vi "Create Runtime.vi"(8 "error in (no error)":errorcluster, 11 "CIF_Iceoryx_PCAP_Universal in":refnum<class "CIF_Iceoryx_PCAP_Universal.lvclass">) -> (0 "error out":errorcluster, 3 "CIF_Iceoryx_PCAP_Universal out":refnum<class "CIF_Iceoryx_PCAP_Universal.lvclass">)   [LabVIEW 2021, in "CIF_Iceoryx_PCAP_Universal.lvclass"]
doc: "To support reconfiguration for different sizes or queue depths, the publisher will register but not create the underlying Iceoryx FIFO. Instead the creation is delayed and is created at run-time. This function is called for each channel on prepare and when a subscriber connects."
uses:
  CIF_Iceoryx_PCAP_Universal.lvclass
  D:/dev/Packages/CIF_Channels_Core/src/CIFChannels/CIFChannels.lvclass
  CIFChannels/CIFChannels.lvclass/CIFChannels.ctl
  ChannelCommon/typedef/Direction.ctl
  ChannelCommon/typedef/Channel State.ctl
  CIF_Iceoryx_PCAP_Universal.lvclass/CIF_Iceoryx_PCAP_Universal.ctl
  <vilib>/CIF Foundation/CIF Iceoryx/typedef/CIF Pcap Publisher Configuration.ctl
  CIFChannels/Accessors/Write Channel State.vi
  CIFChannels/Accessors/Read Name.vi
  CIFChannels/Accessors/Read Direction.vi
  CIFChannels/Accessors/Read Channel State.vi
  <vilib>/CIF Foundation/CIF Iceoryx/SubVIs/Get Path.vi
  <vilib>/CIF Foundation/CIF Iceoryx/SubVIs/Convert Error.vi
  <vilib>/CIF Foundation/CIF Iceoryx/SubVIs/Add Error.vi
  <vilib>/CIF Foundation/CIF Iceoryx/Refnum/CIF Publisher to Refnum.vi
  <vilib>/Utility/error.llb/Trim Whitespace.vi
  <vilib>/CIF Foundation/CIF Iceoryx/SubVIs/Add Error Core.vi
  <vilib>/CIF Foundation/CIF Iceoryx/SubVIs/Convert Error Core.vi
  <vilib>/CIF Foundation/CIF Iceoryx/Iceoryx.lvlib
  ChannelCommon/ChannelCommon.lvlib
  Iceorxy Utilities/Iceoryx Channel Utilities.lvlib
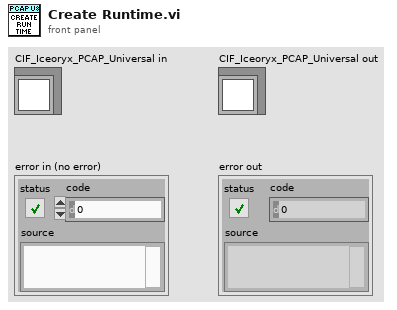
[diagram p1: front panel]
types:
  T1 = typedef "ChannelCommon.lvlib/Direction.ctl" = enum8{"Publisher", "Subscriber"}
  T2 = typedef "ChannelCommon.lvlib/Channel State.ctl" = enum8{"Creating", "Disconnected", "Connecting", "Connected", "Destroyed"}
  T3 = typedef "Iceoryx.lvlib/CIF Pcap Publisher Configuration.ctl" = cluster{"Name":string, "Topic":string, "Link Type":u32, "Descriptor":string, "Max Bytes":u32, "Best Effort Subscribers":u32, "Backpressure Subscribers":u32, "Best Effort Queue Depth":u32, "Backpressure Queue Depth":u32}
  T4 = typedef "Iceoryx.lvlib/CIF Publisher Refnum.ctl" = cluster{"refnum":u64, "CIF Pub":enum8{"cifpub"}}
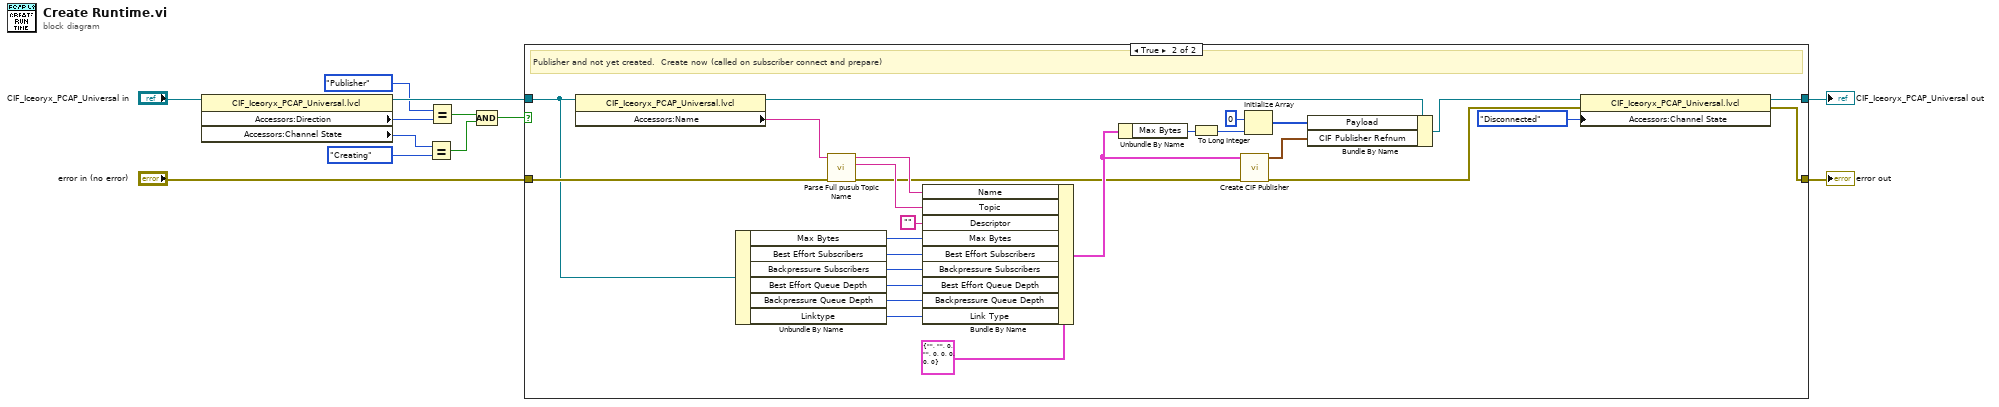
[diagram p0: block diagram]
diagram:
  n1 = property class="CIF_Iceoryx_PCAP_Universal.lvcl"(reference="CIF_Iceoryx_PCAP_Universal in") -> (reference out=w8:refnum<class "CIF_Iceoryx_PCAP_Universal.lvclass">, "Accessors:Direction"=w5:T1, "Accessors:Channel State"=w7:T2)  [unwired: 1 in, 1 out]
  n2 = Equal?(x=w7, y=Channel_State."Creating") -> (x = y?=w3:bool)
  n3 = Equal?(x=Direction."Publisher", y=w5) -> (x = y?=w2:bool)
  n4 = Compound Arithmetic op=AND(w2, w3) -> (w1:bool)
  n5 = case shown="True" w1 {
    tunnel: [w14 w32] -> w12
    tunnel: [w13 w31] -> w11
    tunnel: "error in (no error)" -> [w13 w23]
    tunnel: w8 -> [w14 w15]
    frame False {
    }
    frame True {
      # "Publisher and not yet created.  Create now (called on subscriber connect and prepare)"
      n6 = property class="CIF_Iceoryx_PCAP_Universal.lvcl"(reference=w15) -> (reference out=w25:refnum<class "CIF_Iceoryx_PCAP_Universal.lvclass">, "Accessors:Name"=w24:string)  [unwired: 1 in, 1 out]
      n7 = Unbundle By Name(w15) -> ("Max Bytes"=w22:u32, "Best Effort Subscribers"=w27:u32, "Backpressure Subscribers"=w26:u32, "Best Effort Queue Depth"=w21:u32, "Backpressure Queue Depth"=w20:u32, "Linktype"=w19:u32)
      n8 = call "Parse Full pusub Topic Name.vi"("error in"=w23, "Full pubsub Topic Name"=w24) -> ("error out"=w16:errorcluster, "Topic"=w28:string, "Plugin name"=w29:string)  [unwired: 7 in]
      n9 = Bundle By Name(cluster=T3 {"Name"="", "Topic"="", "Link Type"=0, "Descriptor"="", "Max Bytes"=0, "Best Effort Subscribers"=0, "Backpressure Subscribers"=0, "Best Effort Queue Depth"=0, "Backpressure Queue Depth"=0} ("CIF Pcap Publisher Configuration"), "Name"=w29, "Topic"=w28, "Descriptor"="", "Max Bytes"=w22, "Best Effort Subscribers"=w27, "Backpressure Subscribers"=w26, "Best Effort Queue Depth"=w21, "Backpressure Queue Depth"=w20, "Link Type"=w19) -> (w17:T3)
      n10 = Unbundle By Name(w17) -> ("Max Bytes"=w40:u32)
      n11 = To Long Integer(number=w40) -> (32bit integer=w36:i32)
      n12 = call <vilib>:"Create CIF Publisher.vi"("error in (no error)"=w16, "CIF Pcap Publisher Configuration"=w17) -> ("error out"=w33:errorcluster, "CIF Publisher Refnum"=w39:T4)  [unwired: 8 in]
      n13 = Initialize Array(u8 0 ("Numeric"), w36) -> (w38:u8[])
      n14 = Bundle By Name(cluster=w25, "Payload"=w38, "CIF Publisher Refnum"=w39) -> (w34:refnum<class "CIF_Iceoryx_PCAP_Universal.lvclass">)
      n15 = property class="CIF_Iceoryx_PCAP_Universal.lvcl"(reference=w34, error in=w33, "Accessors:Channel State"=Channel_State."Disconnected" ("Channel State")) -> (reference out=w32:refnum<class "CIF_Iceoryx_PCAP_Universal.lvclass">, error out=w31:errorcluster)
    }
  }
  "CIF_Iceoryx_PCAP_Universal out" <- w12
  "error out" <- w11
